vi "Query Generation Status.vi"(8 "error in (no error)":errorcluster, 11 "AudioGeneration in":refnum<class "AudioGeneration.lvclass">) -> (0 "error out":errorcluster, 1 "generation type":T1, 2 "status":T2, 3 "AudioGeneration out":refnum<class "AudioGeneration.lvclass">, 4 "timeout":bool)   [LabVIEW 2021, in "AudioGeneration.lvclass"]
uses:
  AudioGeneration.lvclass
  controls/generation status.ctl
  controls/generation type.ctl
  controls/generation type and status.ctl
  <vilib>/NI/STM/TCP/Write Message (TCP).vi
  AudioGeneration.lvclass/AudioGeneration.ctl
  <vilib>/NI/STM/NI STM.lvlib
  controls/AudioGenTypeDefs.lvlib
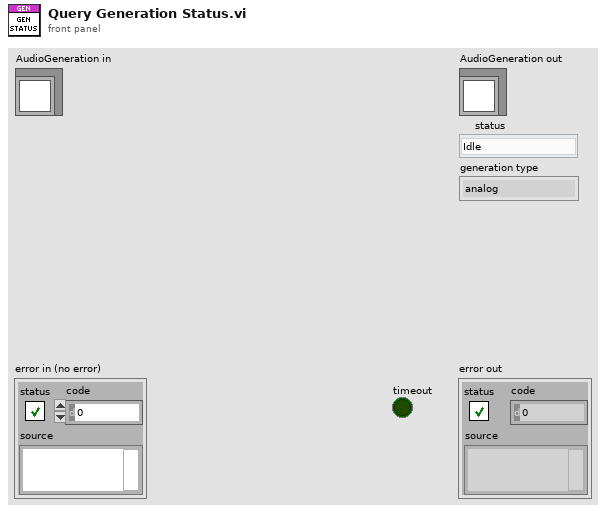
[diagram p1: front panel]
types:
  T1 = typedef "AudioGenTypeDefs.lvlib/generation type.ctl" = enum16{"analog", "digital"}
  T2 = typedef "AudioGenTypeDefs.lvlib/generation status.ctl" = enum16{"Idle", "Committed", "Active"}
  T3 = typedef "AudioGenTypeDefs.lvlib/generation type and status.ctl" = cluster{"status":T2, "generation type":T1}
  T4 = typedef "NI STM.lvlib/TCP Connection Info.ctl" = cluster{"connection ID":refnum<k5>, "meta data":T5[]}
  T5 = typedef "NI STM.lvlib/MetaDataElement.ctl" = string
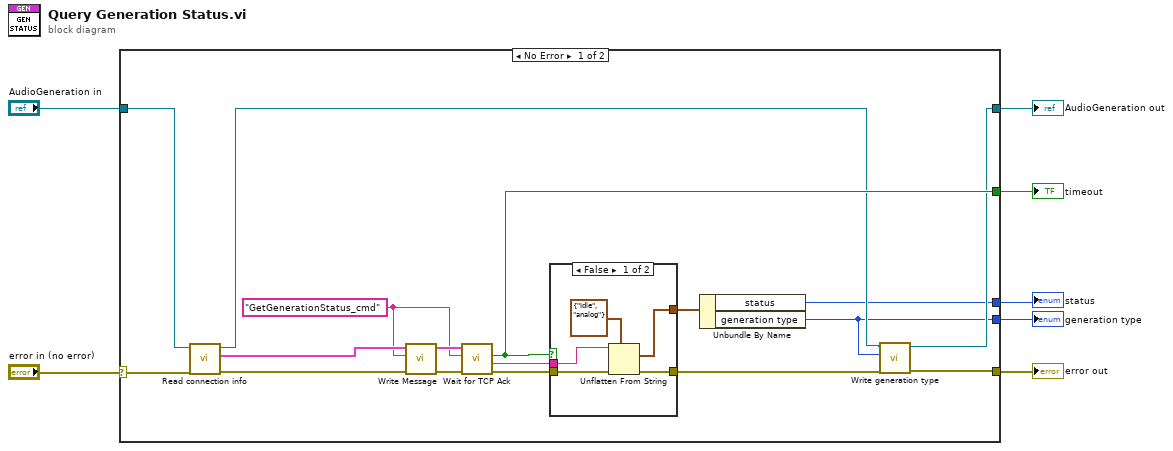
[diagram p0: block diagram]
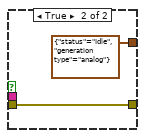
[diagram p2: hidden frame]
diagram:
  n1 = case shown="No Error" "error in (no error)" {
    selector: "error in (no error)" -> [w15 w33]
    tunnel: [w13 w33] -> w6
    tunnel: [w11 w32] -> w5
    tunnel: "AudioGeneration in" -> [w16 w32]
    tunnel: [w17 _] -> w3
    tunnel: [w9 _] -> w2
    tunnel: [w8 _] -> w1
    frame No Error {
      w20 = "GetGenerationStatus_cmd"
      n2 = call-dynamic "Read connection info.vi"("error in (no error)"=w15, "AudioGeneration in"=w16) -> ("error out"=w24:errorcluster, "connection info"=w23:T4, "AudioGeneration out"=w12:refnum<class "AudioGeneration.lvclass">)  [unwired: 7 in]
      n3 = call-poly <vilib>:"Write Message.vi"("error in"=w24, "name"=w20, "connection info in"=w23) -> ("error out"=w22:errorcluster, "connection info out"=w21:T4)  [unwired: 7 in]
      n4 = call "Wait for TCP Ack.vi"("error in (no error)"=w22, "cmd name"=w20, "connection info in"=w21) -> ("error out"=w18:errorcluster, "data string"=w19:string, "timeout"=w17:bool)  [unwired: 5 in, 1 out]
      n5 = case shown="False" w17 {
        tunnel: w19 -> [w28 _]
        tunnel: w18 -> [w29 w31]
        tunnel: [w27 w31] -> w14
        tunnel: [w26 T3 {"status"=enum."Idle", "generation type"=enum."analog"} ("generation")] -> w10
        frame False {
          n6 = Unflatten From String(type=T3 {"status"=enum."Idle", "generation type"=enum."analog"} ("generation"), binary string=w28, error in (no error)=w29) -> (value=w26:T3, error out=w27:errorcluster)  [unwired: 2 in, 1 out]
        }
        frame True {
        }
      }
      n7 = Unbundle By Name(w10) -> ("status"=w9:T2, "generation type"=w8:T1)
      n8 = call-dynamic "Write generation type.vi"("error in (no error)"=w14, "generation type"=w8, "AudioGeneration in"=w12) -> ("error out"=w13:errorcluster, "AudioGeneration out"=w11:refnum<class "AudioGeneration.lvclass">)  [unwired: 7 in]
    }
    frame Error {
    }
  }
  "error out" <- w6
  "AudioGeneration out" <- w5
  "timeout" <- w3
  "status" <- w2
  "generation type" <- w1
